vi "serialization tests.vi"() -> (0 "serialization error":errorcluster, 1 "validation error":errorcluster, 3 "modules OK":bool)   [LabVIEW 2013, in "Profibus Module tests.lvlib"]
uses:
  Profibus Module tests.lvlib
  configuration/Profibus Module configuration.lvclass
  configuration/Profibus Module configuration.lvclass/Profibus Module configuration.ctl
  configuration/Read profibus channels.vi
  configuration/Read byte orders.vi
  configuration/Read slave diagnostics.vi
  configuration/Read RIO interface.vi
  channel/Profibus channel.lvclass
  <vilib>/NI/Tag Bus Module Framework/channel/TBM channel.lvclass
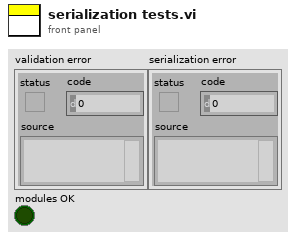
[diagram p1: front panel]
types:
  T1 = typedef "Profibus Module configuration.lvclass/endianness setting.ctl" = cluster{"slave":i8, "big endian":bool}
  T2 = typedef "Profibus Module configuration.lvclass/slave diagnostic configuration.ctl" = cluster{"slave":i8, "report":bool, "channel":refnum<class "TBM channel.lvclass">, "error specs":T3[]}
  T3 = typedef "Profibus Module configuration.lvclass/error throw specification.ctl" = cluster{"byte":i32, "bit":i32, "inverted?":bool, "error":i32}
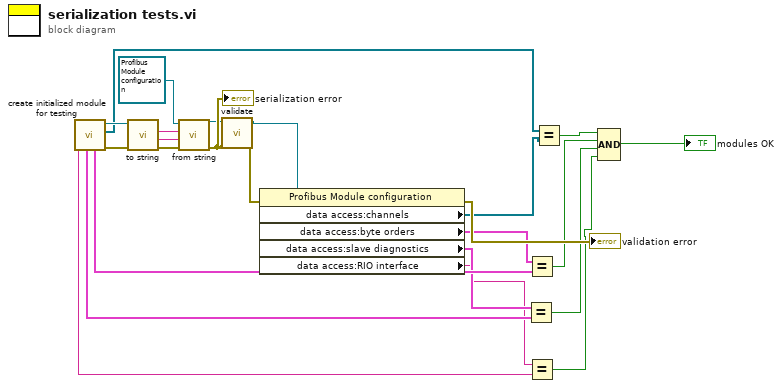
[diagram p0: block diagram]
diagram:
  n1 = call "create initialized module for testing.vi"() -> ("error out"=w18:errorcluster, "1d channels"=w15:refnum<class "Profibus channel.lvclass">[], "Profibus Module configuration out"=w19:refnum<class "Profibus Module configuration.lvclass">, "byte orders"=w11:T1[], "slave diagnostics"=w10:T2[], "RIO interface"=w6:string)  [unwired: 3 in, 3 out]
  n2 = call-dynamic "to string.vi"("error in"=w18, "Profibus Module configuration in"=w19) -> ("error out"=w24:errorcluster, "data"=w23:string, "version"=w22:string)  [unwired: 6 in, 1 out]
  n3 = call-dynamic "from string.vi"("error in"=w24, "data"=w23, "version"=w22, "Profibus Module configuration in"=refnum<class "Profibus Module configuration.lvclass"> refnum ("tag bus configurable plugin module configuration")) -> ("error out"=w4:errorcluster, "Profibus Module configuration out"=w3:refnum<class "Profibus Module configuration.lvclass">)  [unwired: 6 in]
  "serialization error" <- w4
  n4 = call-dynamic "validate.vi"("error in"=w4, "Profibus Module configuration in"=w3) -> ("error out"=w1:errorcluster, "Profibus Module configuration out"=w2:refnum<class "Profibus Module configuration.lvclass">)  [unwired: 8 in]
  n5 = property class="Profibus Module configuration"(reference=w2, error in=w1) -> (error out=→"validation error":errorcluster, "data access:channels"=w14:refnum<class "Profibus channel.lvclass">[], "data access:byte orders"=w8:T1[], "data access:slave diagnostics"=w9:T2[], "data access:RIO interface"=w7:string)  [unwired: 1 out]
  n6 = Equal?(x=w9, y=w10) -> (x = y?=w12:bool)
  n7 = Equal?(x=w8, y=w11) -> (x = y?=w13:bool)
  n8 = Equal?(x=w7, y=w6) -> (x = y?=w5:bool)
  n9 = Equal?(x=w15, y=w14) -> (x = y?=w21:bool)
  n10 = Compound Arithmetic op=AND(w21, w13, w12, w5) -> (→"modules OK":bool)
